vi "breakpoints and other debugging techniques.vi"() -> ()   [LabVIEW 2018]
panel:
  in  "x 3":dbl
  in  "x 2":dbl
  in  "y 2":dbl
  out "x-y":dbl
  in  "x":dbl
  in  "x":dbl
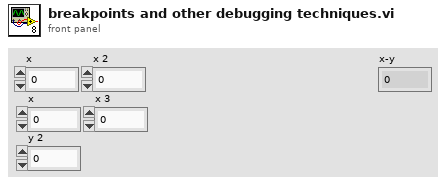
[diagram p1: front panel]
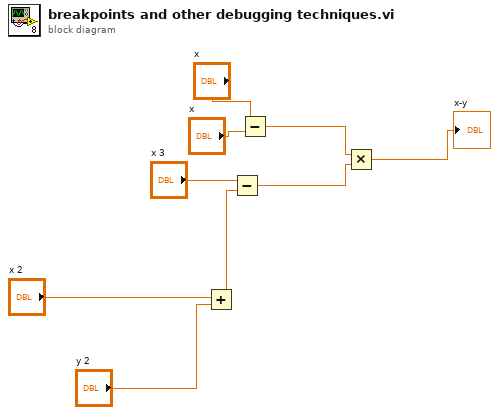
[diagram p0: block diagram]
diagram:
  n1 = Add(x="x 2", y="y 2") -> (x+y=w5:dbl)
  n2 = Subtract(x="x 3", y=w5) -> (x-y=w6:dbl)
  n3 = Subtract(x="x", y="x") -> (x-y=w7:dbl)
  n4 = Multiply(x=w7, y=w6) -> (x*y=→"x-y":dbl)
